vi "Parse Recall Param.vi"(8 "error in (no error)":errorcluster caption="에러 입력(에러 없음)", 10 "JSON string":string, 11 "Instrument Manager 입력":refnum<class "Instrument Manager.lvclass">) -> (0 "error out":errorcluster caption="에러 출력", 1 "Recall Name":string, 2 "Recall Param":T1, 3 "Instrument Manager 출력":refnum<class "Instrument Manager.lvclass">)   [LabVIEW 2023, in "Instrument Manager.lvclass"]
uses:
  Instrument Manager.lvclass
  Param Definition/Recall Param.ctl
  Instrument Manager.lvclass/Instrument Manager.ctl
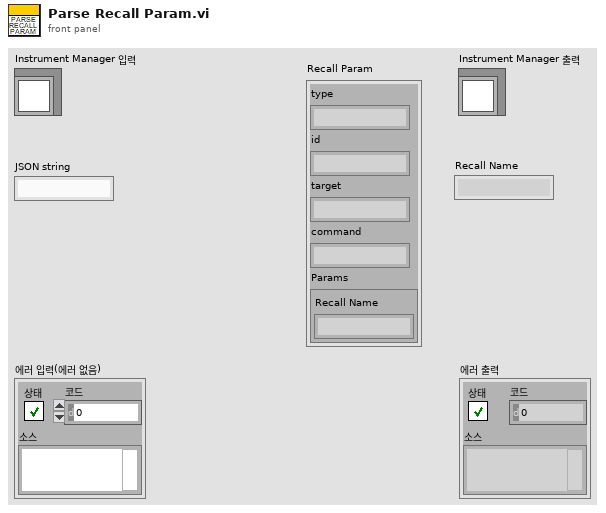
[diagram p1: front panel]
types:
  T1 = typedef "Instrument Manager.lvclass/Recall Param.ctl" = cluster{"type":string, "id":string, "target":string, "command":string, "Params":cluster{"Recall Name":string}}
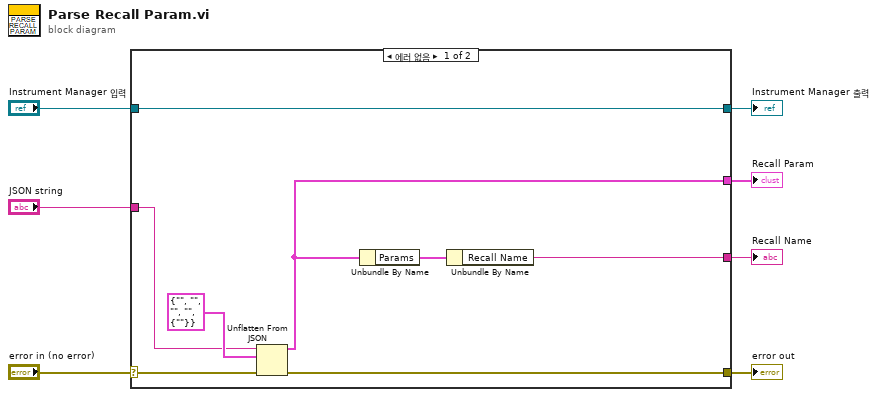
[diagram p0: block diagram]
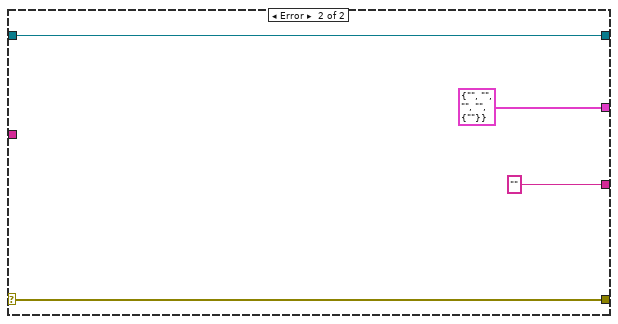
[diagram p2: hidden frame]
diagram:
  n1 = case shown="에러 없음" "error in (no error)" {
    selector: "error in (no error)" -> [w13 w19]
    tunnel: [w12 w19] -> w6
    tunnel: [w15 w18] -> w4
    tunnel: "Instrument Manager 입력" -> [w15 w18]
    tunnel: [w11 T1 {"type"="", "id"="", "target"="", "command"="", "Params"={"Recall Name"=""}} ("Recall Param")] -> w3
    tunnel: [w9 "" ("Recall Name")] -> w2
    tunnel: "JSON string" -> [w8 _]
    frame No Error {
      n2 = Unflatten From JSON(JSON string=w8, type and defaults=T1 {"type"="", "id"="", "target"="", "command"="", "Params"={"Recall Name"=""}} ("Recall Param"), error in (no error)=w13) -> (value=w11:T1, error out=w12:errorcluster)  [unwired: 4 in]
      n3 = Unbundle By Name(w11) -> ("Params"=w10:cluster{"Recall Name":string})
      n4 = Unbundle By Name(w10) -> ("Recall Name"=w9:string)
    }
    frame Error {
    }
  }
  "error out" <- w6
  "Instrument Manager 출력" <- w4
  "Recall Param" <- w3
  "Recall Name" <- w2
